vi "Measurement Logic.vi"(8 "error in":errorcluster, 9 "measurement configuration":T2={"INTERFACE NAME CAN"="Lorem ipsum dolor sit", "IO Mode CAN"=enum."CAN FD", "FD ISO Mode CAN"=enum."Non-ISO", "Termination CAN"=TRUE, "Baudrate CAN"=64, "FD Baudrate CAN"=64, "INTERFACE NAME LIN"="", "Termination LIN"=TRUE, "CAN interface"="", "LIN interface"="", "Network"="", "Baudrate LIN"=0} {"Baudrate CAN" format="%x"}, 10 "measure call context in":refnum<class "Measure Call Context.lvclass">, 11 "Stop OOB Server UE":refnum<user-event>) -> (0 "error out":errorcluster, 1 "measurement results":T1 {"Payload LIN" format="%x"; "DLC LIN" format="%x"; "ID LIN" format="%x"; "Payload CAN" format="%x"; "ID CAN" format="%x"}, 2 "measure call context out":refnum<class "Measure Call Context.lvclass">)   [LabVIEW 2025, in "CAN-LIN Frame Generator.lvclass"]
doc: "Contains the core logic for executing the measurement."
uses:
  CAN-LIN Frame Generator.lvclass
  Measurement Configuration.ctl
  CAN-LIN Frame Generator UI/Toggle.ctl
  Measurement Results.ctl
  <vilib>/Plug-In SDKs/Measurements/Measure Call Context/Measure Call Context.lvclass
  <vilib>/xnet/xnet.llb/XNET Write (Frame LIN).vi
  <vilib>/xnet/xnet.llb/XNET Write (Frame CAN).vi
  OOB Data Transfer/OOB Data Transfer.lvlib
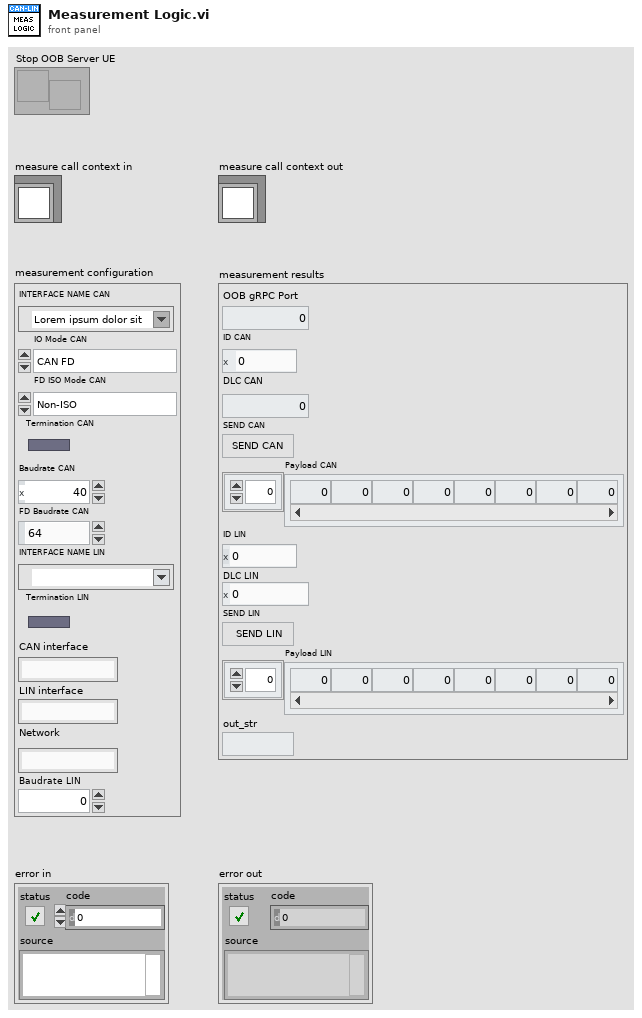
[diagram p1: front panel]
types:
  T1 = typedef "CAN-LIN Frame Generator.lvclass/Measurement Results.ctl" = cluster{"OOB gRPC Port":i32, "ID CAN":u32, "DLC CAN":u32, "SEND CAN":bool, "Payload CAN":u32[], "ID LIN":u32, "DLC LIN":u32, "SEND LIN":bool, "Payload LIN":u32[], "out_str":string}
  T2 = typedef "CAN-LIN Frame Generator.lvclass/Measurement Configuration.ctl" = cluster{"INTERFACE NAME CAN":refnum<k21>, "IO Mode CAN":enum32{"CAN", "CAN FD", "CAN FD + BRS"}, "FD ISO Mode CAN":enum32{"ISO", "Legacy ISO", "Non-ISO"}, "Termination CAN":T3, "Baudrate CAN":u32, "FD Baudrate CAN":u32, "INTERFACE NAME LIN":refnum<k21>, "Termination LIN":T3, "CAN interface":string, "LIN interface":string, "Network":string, "Baudrate LIN":u32}
  T3 = typedef "Toggle.ctl" = bool
  T4 = typedef "OOB Data Transfer.lvlib/OOB to Logic Data.ctl" = cluster{"PauseResume":bool, "Export":string, "ID CAN":u32, "Type CAN":T5, "DLC CAN":u32, "SEND CAN":bool, "Payload CAN":u32[], "ID LIN":u32, "DLC LIN":u32, "SEND LIN":bool, "Payload LIN":u32[], "out_str":string, "cfg err":bool}
  T5 = typedef "XNET Frame Type CAN.ctl" = u8
  T6 = typedef "XNET Frame LIN.ctl" = cluster{"timestamp":timestamp, "payload":u8[], "identifier":u32, "type":T7, "event ID":u8, "event slot?":bool, "echo?":bool}
  T7 = typedef "XNET Frame Type LIN.ctl" = u8
  T8 = typedef "XNET Frame CAN.ctl" = cluster{"timestamp":timestamp, "payload":u8[], "identifier":u32, "type":T5, "extended?":bool, "echo?":bool}
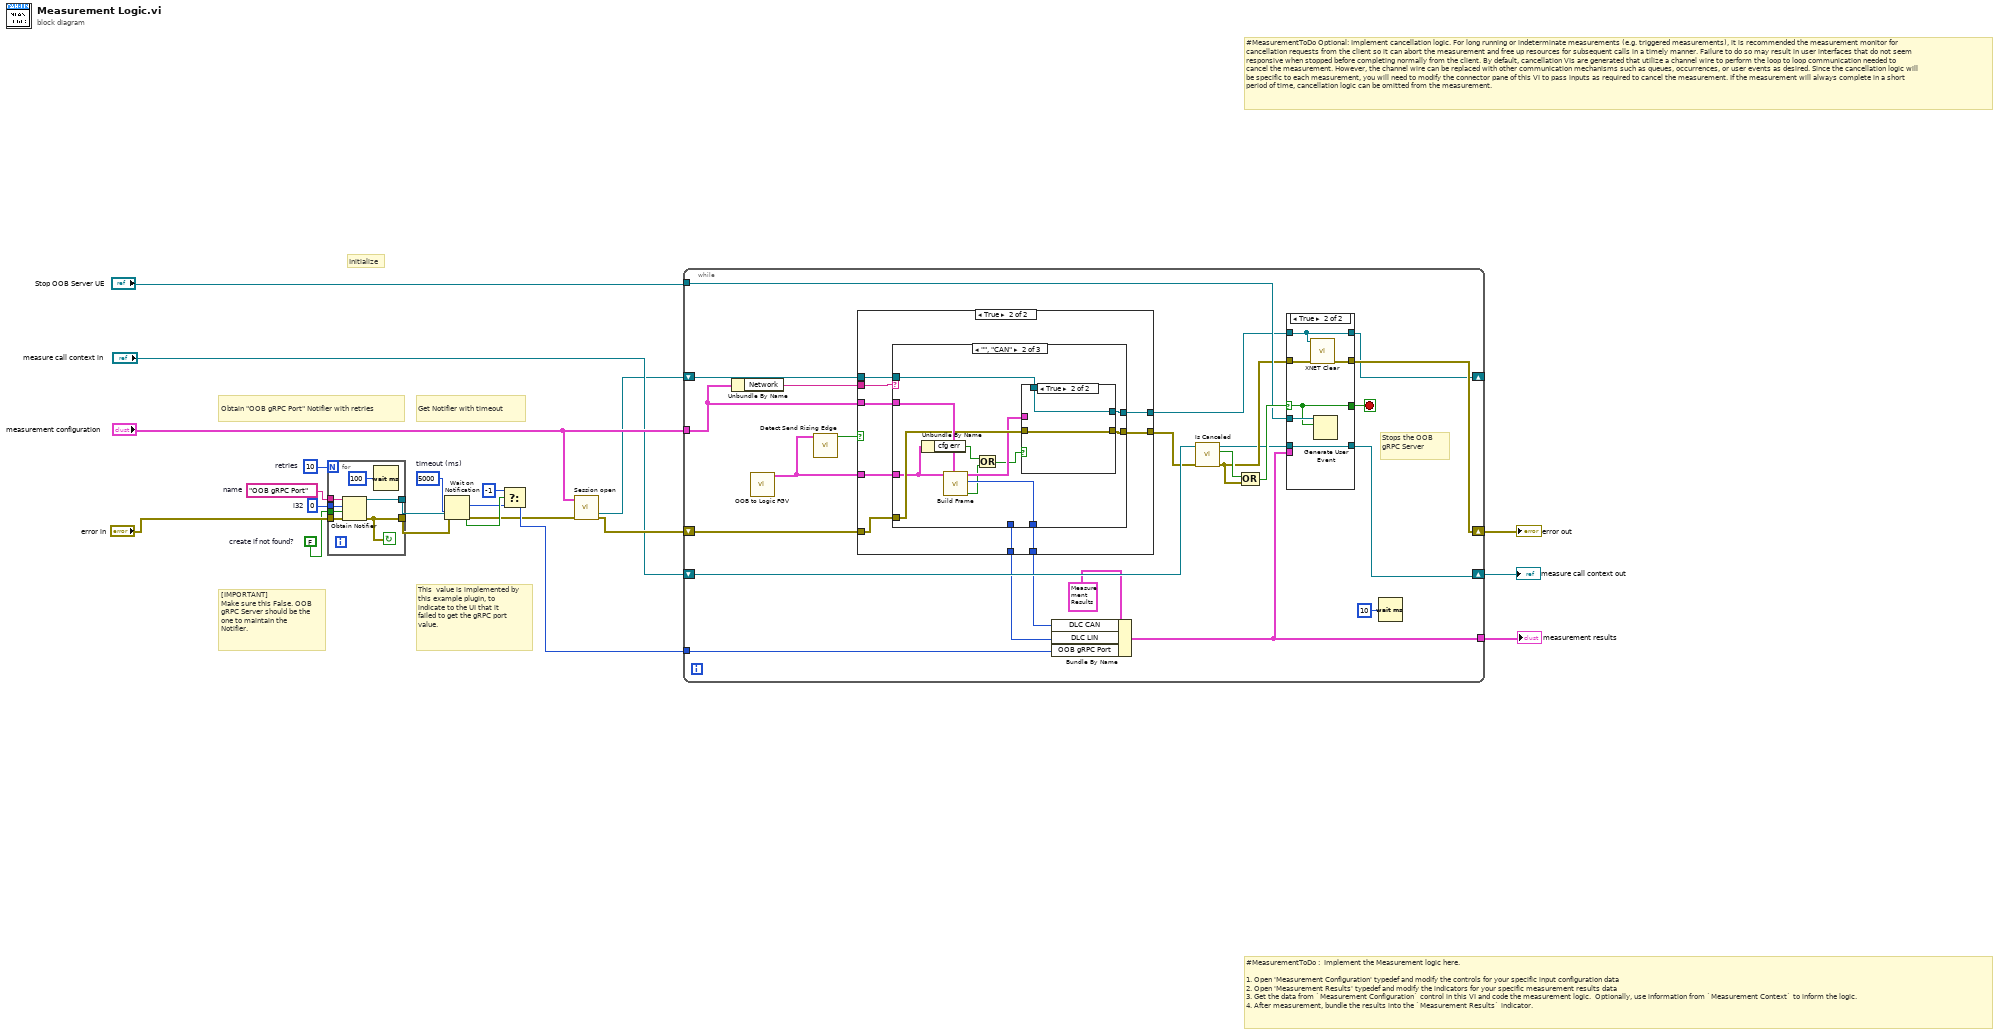
[diagram p0: block diagram]
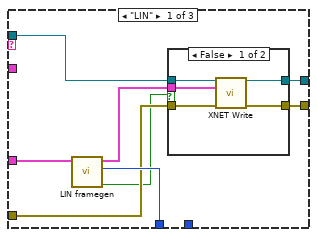
[diagram p3: hidden frame]
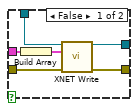
[diagram p5: hidden frame]
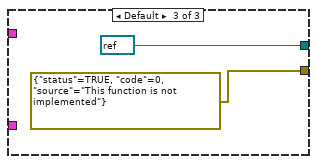
[diagram p6: hidden frame]
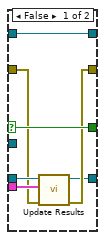
[diagram p7: hidden frame]
diagram:
  w2 = FALSE  # create if not found?
  w7 = 0  # i32
  w6 = "OOB gRPC Port"  # name
  w8 = 10  # retries
  w9 = 5000  # timeout (ms)
  # "This  value is implemented by this example plugin, to indicate to the UI that it failed to get the gRPC port value."
  # "[IMPORTANT] \nMake sure this False. OOB gRPC Server should be the one to maintain the Notifier."
  # "Initialize"
  # "Obtain \"OOB gRPC Port\" Notifier with retries"
  # "Get Notifier with timeout"
  # "#MeasurementToDo Optional: Implement cancellation logic. For long running or indeterminate measurements (e.g. triggered measurements), it is recommended the measurement monitor for cancellation requests from the client so it can abort the measurement and free up resources for subsequent calls in a timely manner. Failure to do so may result in user interfaces that do not seem responsive when stopped before completing normally from the client. By default, cancellation VIs are generated that utilize a channel wire to perform the loop to loop communication needed to cancel the measurement. However, the channel wire can be replaced with other communication mechanisms such as queues, occurrences, or user events as desired. Since the cancellation logic will be specific to each measurement, you will need to modify the connector pane of this VI to pass inputs as required to cancel the measurement. If the measurement will always complete in a short period of time, cancellation logic can be omitted from the measurement."
  # "#MeasurementToDo :  Implement the Measurement logic here.\n\n1. Open 'Measurement Configuration' typedef and modify the controls for your specific input configuration data\n2. Open 'Measurement Results' typedef and modify the indicators for your specific measurement results data\n3. Get the data from `Measurement Configuration` control in this VI and code the measurement logic.  Optionally, use information from `Measurement Context` to inform the logic.\n4. After measurement, bundle the results into the `Measurement Results` indicator."
  n1 = for {
    N: w8 -> [_]
    tunnel: [w26] -> w11
    tunnel: [w28] -> w10
    tunnel: w6 -> [w25]
    tunnel: w7 -> [w24]
    tunnel: "error in" -> [w23]
    tunnel: w2 -> [w22]
    stop <- w26 continue-if-true
    n2 = Obtain Notifier(name (unnamed)=w25, notification data type=w24, create if not found? (T)=w22, error in (no error)=w23) -> (notifier out=w28:refnum<notifier>, error out=w26:errorcluster)  [unwired: 1 out]
    n3 = Wait (ms)(milliseconds to wait=u32 100) -> ()  [unwired: 1 out]
  }
  n4 = Wait on Notification(notifier=w10, timeout in ms (-1)=w9, error in (no error)=w11) -> (notification=w4:i32, timed out?=w5:bool, error out=w1:errorcluster)  [unwired: 1 in, 1 out]
  n5 = Select(t=-1, s=w5, f=w4) -> (s? t:f=w17:i32)
  n6 = call "Session open.vi"("error in"=w1, "measurement configuration"="measurement configuration") -> ("error out"=w19:errorcluster, "session out"=w12:refnum<k21>)  [unwired: 8 in]
  n7 = while {
    tunnel: [w31] -> w21
    tunnel: "measurement configuration" -> [w33]
    tunnel: w17 -> [w51]
    shift-right: [w43] -> w14
    shift-left: w19 -> [w52]
    tunnel: "Stop OOB Server UE" -> [w48]
    shift-right: [w30] -> w13
    shift-left: "measure call context in" -> [w47]
    shift-right: [w41] -> _
    shift-left: w12 -> [w40]
    stop <- w45 stop-if-true
    # "Stops the OOB gRPC Server"
    n8 = Unbundle By Name(w33) -> ("Network"=w39:string)
    n9 = call "OOB to Logic FGV.vi"() -> ("OOB to Logic Data out"=w35:T4)  [unwired: 10 in, 1 out]
    n10 = call "Detect Send Rising Edge.vi"("OOB to Logic Data in"=w35) -> ("crossing"=w29:bool)  [unwired: 10 in]
    n11 = case shown="True" w29 {
      tunnel: w40 -> [w54 w63]
      tunnel: w52 -> [w53 w55]
      tunnel: w39 -> [_ w62]
      tunnel: [w53 w61] -> w46
      tunnel: [w54 w60] -> w42
      tunnel: [_ w59] -> w37
      tunnel: [_ w58] -> w36
      tunnel: w35 -> [_ w57]
      tunnel: w33 -> [_ w56]
      frame False {
      }
      frame True {
        n12 = case shown="\"\", \"CAN\"" w62 {
          tunnel: w63 -> [w71 w87 _]
          tunnel: w55 -> [w65 w86 _]
          tunnel: [w70 w85 errorcluster {"status"=TRUE, "code"=0, "source"="This function is not implemented"} ("error out")] -> w61
          tunnel: [_ w89 _] -> w59
          tunnel: [w66 _ _] -> w58
          tunnel: [w68 w84 refnum<k21> refnum ("session out")] -> w60
          tunnel: w57 -> [w67 w80 _]
          tunnel: w56 -> [_ w88 _]
          frame "LIN" {
            n13 = call "LIN framegen.vi"("OOB to Logic Data in"=w67) -> ("err"=w64:bool, "DLC 2"=w66:u32, "Array"=w69:T6[])  [unwired: 8 in]
            n14 = case shown="False" w64 {
              tunnel: w71 -> [w76 w78]
              tunnel: [w75 w77] -> w70
              tunnel: w69 -> [w74 _]
              tunnel: [w73 w78] -> w68
              tunnel: w65 -> [w72 w77]
              frame False {
                n15 = call-poly <vilib>:"XNET Write.vi"("session in"=w76, "data"=w74, "error in (no error)"=w72) -> ("session out"=w73:refnum<k21>, "error out"=w75:errorcluster)  [unwired: 11 in]
              }
              frame True {
              }
            }
          }
          frame "", "CAN" {
            n16 = Unbundle By Name(w80) -> ("cfg err"=w79:bool)
            n17 = call "Build Frame.vi"("measurement configuration"=w88, "OOB to Logic Data in"=w80) -> ("err"=w82:bool, "DLC out"=w89:u32, "output cluster"=w83:T8)  [unwired: 7 in]
            n18 = Or(x=w79, y=w82) -> (x .or. y?=w81:bool)
            n19 = case shown="True" w81 {
              tunnel: w87 -> [w95 w97]
              tunnel: w86 -> [w93 w96]
              tunnel: [w92 w96] -> w85
              tunnel: [w91 w97] -> w84
              tunnel: w83 -> [w90 _]
              frame False {
                n20 = Build Array(w90) -> (w94:T8[])
                n21 = call-poly <vilib>:"XNET Write.vi"("session in"=w95, "data"=w94, "error in (no error)"=w93) -> ("session out"=w91:refnum<k21>, "error out"=w92:errorcluster)  [unwired: 11 in]
              }
              frame True {
              }
            }
          }
          frame Default {
          }
        }
      }
    }
    n22 = Bundle By Name(cluster=T1 {"OOB gRPC Port"=0, "ID CAN"=0, "DLC CAN"=0, "SEND CAN"=FALSE, "Payload CAN"=[0, 0, 0, 0, 0, 0, 0, 0, 0, 0, 0, 0, 0, 0, 0, 0, 0, 0, 0, 0, 0, 0, 0, 0, 0, 0, 0, 0, 0, 0, 0, 0, 0, 0, 0, 0, 0, 0, 0, 0, 0, 0, 0, 0, 0, 0, 0, 0, 0, 0, 0, 0, 0, 0, 0, 0, 0, 0, 0, 0, 0, 0, 0, 0], "ID LIN"=0, "DLC LIN"=0, "SEND LIN"=FALSE, "Payload LIN"=[0, 0, 0, 0, 0, 0, 0, 0], "out_str"=""} ("Measurement Results"), "DLC CAN"=w37, "DLC LIN"=w36, "OOB gRPC Port"=w51) -> (w31:T1)
    n23 = call <vilib>:"Is Canceled.vi"("error in"=w46, "measure call context in"=w47) -> ("error out"=w44:errorcluster, "is canceled?"=w50:bool, "measure call context out"=w32:refnum<class "Measure Call Context.lvclass">)  [unwired: 7 in]
    n24 = Compound Arithmetic op=OR(w50, w44) -> (w49:bool)
    n25 = case shown="True" w49 {
      selector: w49 -> [w106 w111]
      tunnel: w48 -> [_ w112]
      tunnel: [w106 w111] -> w45
      tunnel: w44 -> [w102 w110]
      tunnel: [w101 w109] -> w43
      tunnel: w42 -> [w105 w108]
      tunnel: [w105 w108] -> w41
      tunnel: w32 -> [w104 w107]
      tunnel: w31 -> [w103 _]
      tunnel: [w100 w107] -> w30
      frame False {
        n26 = call <vilib>:"Update Results.vi"("error in"=w102, "measurement results"=w103, "measure call context in"=w104) -> ("error out"=w101:errorcluster, "measure call context out"=w100:refnum<class "Measure Call Context.lvclass">)  [unwired: 7 in]
      }
      frame True {
        n27 = call <vilib>:"XNET Clear.vi"("session in"=w108, "error in (no error)"=w110) -> ("error out"=w109:errorcluster)  [unwired: 13 in]
        n28 = Generate User Event(user event=w112, event data cluster=w111) -> ()  [unwired: 2 in, 2 out]
      }
    }
    n29 = Wait (ms)(milliseconds to wait=u32 10) -> ()  [unwired: 1 out]
  }
  "error out" <- w14
  "measurement results" <- w21
  "measure call context out" <- w13
